vi "Light_Monitor.vi"() -> ()   [LabVIEW 2026]
panel:
  out "연결·측정 상태":string
  in  "측정중지":bool
  in  "측정시작":bool
  out "CSV 저장오류":errorcluster
  out "마지막오류":errorcluster
  in  "CSV 저장 폴더":path
  out "ADC Raw":dbl
  in  "연결종료":bool
  out "Waveform Chart":i32(graph)
  out "Received JSON":string
  in  "port":dbl
  in  "pi_IP":string
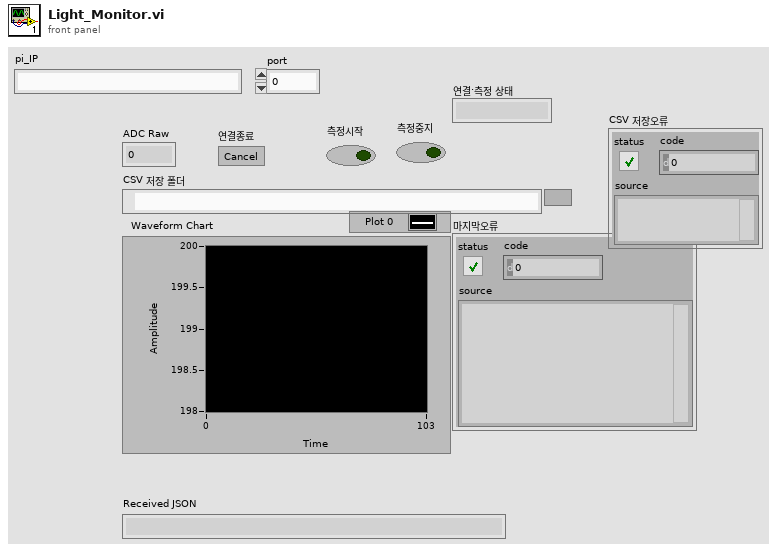
[diagram p1: front panel]
types:
  T1 = enum16{"Running", "Stopped", "WaitStartAck", "WaitStopAck"}
  T2 = enum16{"open", "replace", "create", "open or create", "replace or create", "replace or create with confirmation"}
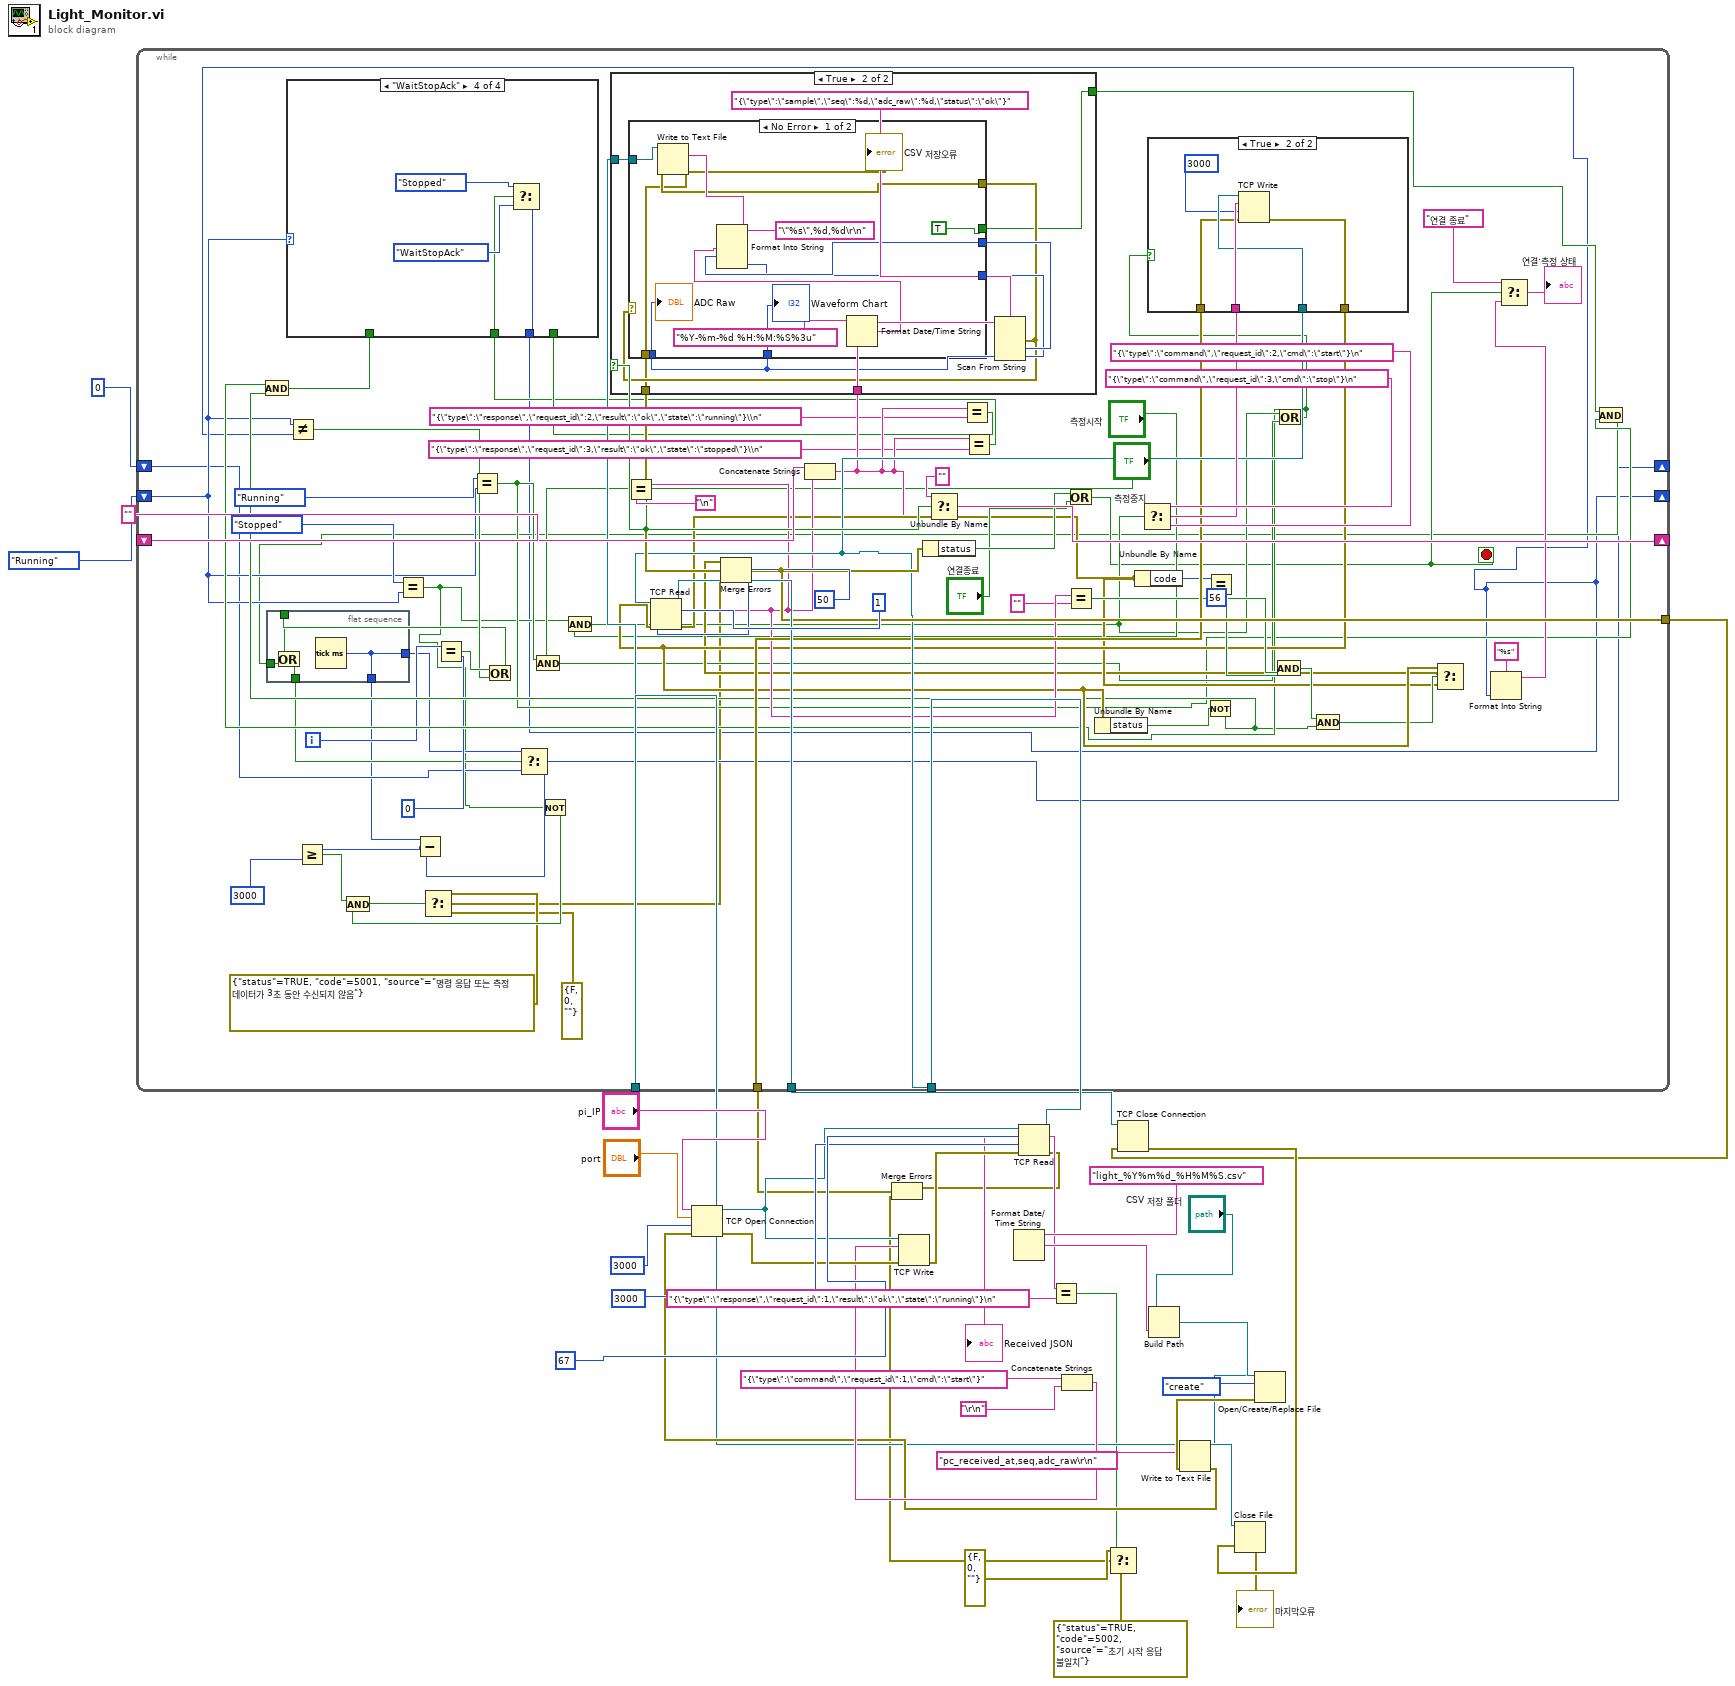
[diagram p0: block diagram]
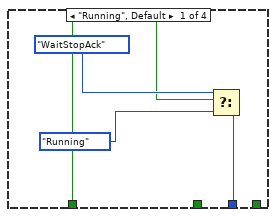
[diagram p2: hidden frame]
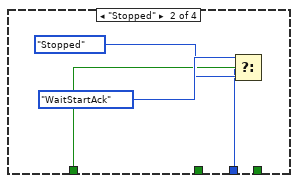
[diagram p3: hidden frame]
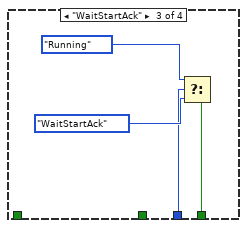
[diagram p4: hidden frame]
diagram:
  n1 = Format Date/Time String(time format string (%c)="light_%Y%m%d_%H%M%S.csv") -> (date/time string=w21:string)  [unwired: 2 in]
  n2 = Concatenate Strings "Concatenate Strings"("{\"type\":\"command\",\"request_id\":1,\"cmd\":\"start\"}", "\r\n") -> (w27:string)
  n3 = Build Path(base path="CSV 저장 폴더", name or relative path=w21) -> (appended path=w20:path)
  n4 = Open/Create/Replace File(file path (use dialog)=w20, operation (0:open)=T2."create") -> (refnum out=w12:refnum<file>, error out=w18:errorcluster)  [unwired: 4 in, 1 out]
  n5 = Write to Text File(file (use dialog)=w12, text="pc_received_at,seq,adc_raw\r\n", error in=w18) -> (refnum out=w15:refnum<file>, error out=w16:errorcluster)  [unwired: 1 in, 1 out]
  n6 = TCP Open Connection(address="pi_IP", remote port or service name="port", timeout ms (60000)=3000, error in (no error)=w16) -> (connection ID=w32:refnum<k5>, error out=w31:errorcluster)  [unwired: 1 in]
  n7 = TCP Write(connection ID=w32, data in=w27, error in (no error)=w31) -> (error out=w30:errorcluster)  [unwired: 1 in, 2 out]
  n8 = TCP Read(connection ID=w32, bytes to read=67, error in (no error)=w30, 9:3000) -> (connection ID out=w26:refnum<k5>, data out=w8:string, error out=w3:errorcluster)  [unwired: 1 in]
  "Received JSON" <- w8
  n9 = Equal?(x=w8, y="{\"type\":\"response\",\"request_id\":1,\"result\":\"ok\",\"state\":\"running\"}\n") -> (x = y?=w6:bool)
  n10 = Select(t=errorcluster {"status"=FALSE, "code"=0, "source"=""} ("error constant"), s=w6, f=errorcluster {"status"=TRUE, "code"=5002, "source"="초기 시작 응답 불일치"}) -> (s? t:f=w1:errorcluster)
  n11 = Merge Errors(w3, w1) -> (w2:errorcluster)
  n12 = while {
    tunnel: w26 -> [w94]
    tunnel: [w108] -> w25
    tunnel: w2 -> [w93]
    tunnel: [w98] -> w11
    shift-right: [w105] -> _
    shift-left: "" -> [w107]
    tunnel: w12 -> [w100]
    shift-right: [w38] -> _
    shift-left: T1."Running" -> [w59]
    shift-right: [w48] -> _
    shift-left: u32 0 -> [w50]
    i -> [w58]
    stop <- w63 stop-if-true
    n13 = flat-sequence {
      tunnel: w54 -> [w114]
      tunnel: w53 -> [w113]
      tunnel: [w112] -> w52
      tunnel: [w111] -> w51
      tunnel: [w111] -> w49
      frame #0 {
        n14 = Or(x=w113, y=w114) -> (x .or. y?=w112:bool)
        n15 = Tick Count (ms)() -> (millisecond timer value=w111:u32)
      }
    }
    n16 = Equal?(x=T1."Stopped", y=w59) -> (x = y?=w45:bool)
    n17 = Equal?(x=w58, y=0) -> (x = y?=w56:bool)
    n18 = Equal?(x=T1."Running", y=w59) -> (x = y?=w60:bool)
    n19 = Select(t=w51, s=w52, f=w50) -> (s? t:f=w48:u32)
    n20 = Subtract(x=w49, y=w48) -> (x-y=w47:u32)
    n21 = Greater Or Equal?(x=w47, y=u32 3000) -> (x >= y?=w44:bool)
    n22 = And(x=w60, y="측정중지") -> (x .and. y?=w73:bool)
    n23 = Not(x=w45) -> (.not. x?=w43:bool)
    n24 = And(x=w44, y=w43) -> (x .and. y?=w42:bool)
    n25 = Select(t=errorcluster {"status"=TRUE, "code"=5001, "source"="명령 응답 또는 측정 데이터가 3초 동안 수신되지 않음"} ("error constant"), s=w42, f=errorcluster {"status"=FALSE, "code"=0, "source"=""}) -> (s? t:f=w39:errorcluster)
    n26 = And(x=w45, y="측정시작") -> (x .and. y?=w72:bool)
    n27 = Select(t="{\"type\":\"command\",\"request_id\":3,\"cmd\":\"stop\"}\n", s=w72, f="{\"type\":\"command\",\"request_id\":2,\"cmd\":\"start\"}\n") -> (s? t:f=w95:string)
    n28 = Or(x=w72, y=w73) -> (x .or. y?=w71:bool)
    n29 = case shown="True" w71 {
      tunnel: w95 -> [_ w136]
      tunnel: w94 -> [_ w135]
      tunnel: w93 -> [w131 w134]
      tunnel: [w131 w133] -> w84
      frame False {
      }
      frame True {
        n30 = TCP Write(connection ID=w135, data in=w136, error in (no error)=w134, 9:3000 ("timeout ms (25000)")) -> (error out=w133:errorcluster)  [unwired: 2 out]
      }
    }
    n31 = TCP Read(connection ID=w94, bytes to read=1, error in (no error)=w84, 9:50) -> (connection ID out=w108:refnum<k5>, data out=w90:string, error out=w82:errorcluster)  [unwired: 1 in]
    n32 = Equal?(x=w90, y="\n") -> (x = y?=w103:bool)
    n33 = Concatenate Strings "Concatenate Strings"(w107, w90) -> (w80:string)
    n34 = case shown="True" w103 {
      tunnel: w80 -> [_ w144]
      tunnel: w100 -> [_ w140]
      tunnel: [_ w138] -> w99
      tunnel: [_ w137] -> w61
      frame False {
      }
      frame True {
        n35 = Scan From String "Scan From String"(format string="{\"type\":\"sample\",\"seq\":%d,\"adc_raw\":%d,\"status\":\"ok\"}", input string=w144) -> (error out=w139:errorcluster, output 1=w142:i32, output 2=w141:i32)  [unwired: 4 in, 2 out]
        n36 = case shown="No Error" w139 {
          tunnel: w141 -> [w156 _]
          tunnel: w141 -> [w155 _]
          tunnel: w142 -> [w151 _]
          tunnel: w141 -> [w150 _]
          tunnel: w140 -> [w149 _]
          tunnel: w139 -> [w147 _]
          tunnel: [w146 _] -> w138
          tunnel: [TRUE _] -> w137
          frame No Error {
            n37 = Format Date/Time String(time format string (%c)="%Y-%m-%d %H:%M:%S%3u") -> (date/time string=w152:string)  [unwired: 2 in]
            n38 = Format Into String "Format Into String"(format string="\"%s\",%d,%d\r\n", w152, w151, w150) -> (resulting string=w148:string)  [unwired: 2 in, 1 out]
            n39 = Write to Text File(file (use dialog)=w149, text=w148, error in=w147) -> (error out=w146:errorcluster)  [unwired: 1 in, 2 out]
            "CSV 저장오류" <- w146
            "Waveform Chart" <- w155
            "ADC Raw" <- w156
          }
          frame Error {
          }
        }
      }
    }
    n40 = Select(t="", s=w103, f=w80) -> (s? t:f=w105:string)
    n41 = Equal?(x=w80, y="{\"type\":\"response\",\"request_id\":2,\"result\":\"ok\",\"state\":\"running\"}\\n") -> (x = y?=w68:bool)
    n42 = Equal?(x=w80, y="{\"type\":\"response\",\"request_id\":3,\"result\":\"ok\",\"state\":\"stopped\"}\\n") -> (x = y?=w67:bool)
    n43 = Equal?(x=w90, y="") -> (x = y?=w86:bool)
    n44 = Unbundle By Name(w84) -> ("status"=w88:bool)
    n45 = Unbundle By Name "Unbundle By Name"(w82) -> ("code"=w92:i32)
    n46 = Not(x=w88) -> (.not. x?=w70:bool)
    n47 = And(x=w71, y=w70) -> (x .and. y?=w69:bool)
    n48 = case shown="\"WaitStopAck\"" w59 {
      tunnel: w69 -> [w116 w120 _ _]
      tunnel: [w115 w119 w123 w127] -> w38
      tunnel: w68 -> [_ _ w124 _]
      tunnel: w67 -> [_ _ _ w128]
      frame "Running", Default {
        n49 = Select(t=T1."WaitStopAck", s=w116, f=T1."Running") -> (s? t:f=w115:T1)
      }
      frame "Stopped" {
        n50 = Select(t=T1."WaitStartAck", s=w120, f=T1."Stopped") -> (s? t:f=w119:T1)
      }
      frame "WaitStartAck" {
        n51 = Select(t=T1."Running", s=w124, f=T1."WaitStartAck") -> (s? t:f=w123:T1)
      }
      frame "WaitStopAck" {
        n52 = Select(t=T1."Stopped", s=w128, f=T1."WaitStopAck") -> (s? t:f=w127:T1)
      }
    }
    n53 = Not Equal?(x=w59, y=w38) -> (x != y?=w55:bool)
    n54 = Or(x=w56, y=w55) -> (x .or. y?=w53:bool)
    n55 = Equal?(x=w92, y=56) -> (x = y?=w87:bool)
    n56 = And(x=w87, y=w86) -> (x .and. y?=w85:bool)
    n57 = And(x=w85, y=w70) -> (x .and. y?=w83:bool)
    n58 = Select(t=w84, s=w83, f=w82) -> (s? t:f=w81:errorcluster)
    n59 = Merge Errors "Merge Errors"(w81, w99, w39) -> (w98:errorcluster)
    n60 = Unbundle By Name "Unbundle By Name"(w98) -> ("status"=w102:bool)
    n61 = Or(x=w102, y="연결종료") -> (x .or. y?=w63:bool)
    n62 = Format Into String "Format Into String"(format string="%s", w38) -> (resulting string=w65:string)  [unwired: 2 in, 1 out]
    n63 = Select(t="연결 종료", s=w63, f=w65) -> (s? t:f=→"연결·측정 상태":string)
    n64 = And(x=w61, y=w60) -> (x .and. y?=w54:bool)
  }
  n65 = TCP Close Connection(connection ID=w25, error in (no error)=w11) -> (error out=w14:errorcluster)  [unwired: 1 in, 1 out]
  n66 = Close File(refnum=w15, error in=w14) -> (error out=→"마지막오류":errorcluster)  [unwired: 1 out]
